vi "OpenG Array filter - Invert Array Template.vi"() -> ()   [LabVIEW 2012]
panel:
  out "filtered item indices":i32[](array[numeric])
  out "filtered array":variant[](array[variant])
  in  "items to filter":variant[](array[variant])
  in  "Array Input":variant[](array[variant])
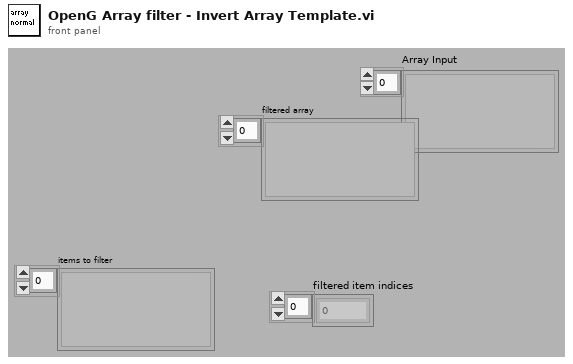
[diagram p1: front panel]
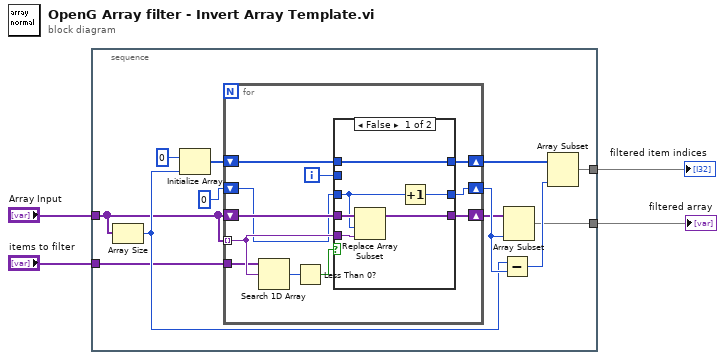
[diagram p0: block diagram]
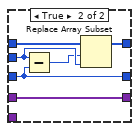
[diagram p2: hidden frame]
diagram:
  n1 = stacked-sequence {
    tunnel: "items to filter" -> [w7]
    tunnel: [w5] -> w3
    tunnel: "Array Input" -> [w8]
    tunnel: [w6] -> w1
    frame #0 {
      n2 = Array Size(array=w8) -> (size(s)=w13:i32)
      n3 = Initialize Array(0 ("Numeric"), w13) -> (w12:i32[])
      n4 = for {
        tunnel: w8 -> [w24] mode=indexing
        shift-right: [w25] -> w10
        shift-left: w8 -> [w27]
        shift-right: [w22] -> w15
        shift-left: 0 -> [w23]
        shift-right: [w19] -> w14
        shift-left: w12 -> [w20]
        tunnel: w7 -> [w18]
        i -> [w17]
        n5 = Search 1D Array(1D array=w18, element=w24) -> (index of element=w21:i32)  [unwired: 1 out]
        n6 = Less Than 0?(x=w21) -> (x < 0?=w26:bool)
        n7 = case shown="False" w26 {
          tunnel: w27 -> [w33 w39]
          tunnel: [w32 w39] -> w25
          tunnel: w24 -> [w31 _]
          tunnel: w23 -> [w29 w35]
          tunnel: [w30 w35] -> w22
          tunnel: w20 -> [w28 w38]
          tunnel: [w28 w37] -> w19
          tunnel: w17 -> [_ w36]
          frame False {
            n8 = Replace Array Subset(array=w33, new element=w31, index=w29) -> (w32:variant[])
            n9 = Increment(x=w29) -> (x+1=w30:i32)
          }
          frame True {
            n10 = Subtract(x=w36, y=w35) -> (x-y=w34:i32)
            n11 = Replace Array Subset(array=w38, new element=w36, index=w34) -> (w37:i32[])
          }
        }
      }
      n12 = Subtract(x=w13, y=w15) -> (x-y=w16:i32)
      n13 = Array Subset(array=w10, length=w15) -> (w6:variant[])  [unwired: 1 in]
      n14 = Array Subset(array=w14, length=w16) -> (w5:i32[])  [unwired: 1 in]
    }
  }
  "filtered array" <- w1
  "filtered item indices" <- w3
